vi "Is Dmtch Completed.vi"(8 "error in (no error)":errorcluster caption="错误输入（无错误）", 11 "uProgress":u32) -> (0 "error out":errorcluster caption="错误输出", 2 "function return":bool, 3 "uProgress out":u32)   [LabVIEW 2017, in "smncsftmt.lvlib"]
doc: "__declspec(dllexport) bool IsDmtchCompleted(unsigned int* uProgress);"
uses:
  smncsftmt.lvlib
  smncsftmt.dll
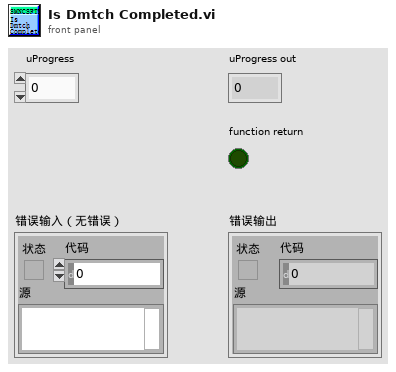
[diagram p1: front panel]
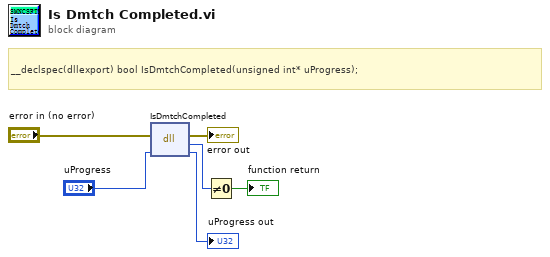
[diagram p0: block diagram]
diagram:
  # "__declspec(dllexport) bool IsDmtchCompleted(unsigned int* uProgress);"
  n1 = dll-call lib="PTH2oabs CUsersaDesktop\nLABVIEW范例National InstrumentsLabVIEW 2017user.lib\tsmncsftmtsmncsftmt.*" fn="IsDmtchCompleted"(error in="error in (no error)", "uProgress"="uProgress") -> (error out=→"error out":errorcluster, w5:u8, "uProgress"=→"uProgress out":u32)  [unwired: 2 in, 1 out]
  n2 = Not Equal To 0?(x=w5) -> (x != 0?=→"function return":bool)
